vi "onDestroy.vi"(8 "error in (no error)":errorcluster, 11 "Pump":refnum<class "Pump.lvclass">) -> (0 "error out":errorcluster, 3 "Pump out":refnum<class "Pump.lvclass">)   [LabVIEW 2014, in "Pump.lvclass"]
doc: "JKI State Machine Objects (SMO) 1.4.0.57\nJKI - JKI\nCopyright (c) 2018, JKI"
uses:
  Pump.lvclass
  Pump.lvclass/Pump.ctl
  <vilib>/JKI/JKI SMO/SMO/SMO.lvclass
panel:
  # "For instructions on how to use the JKI State Machine Objects, examples and video tutorials, visit:\nhttp://jki.net/state-machine-objects/\n\nJKI State Machine Objects™\nhttp://jki.net/state-machine-objects/\nCopyright (C) 2005-2015, JKI <info@jki.net>\nALL RIGHTS RESERVED"
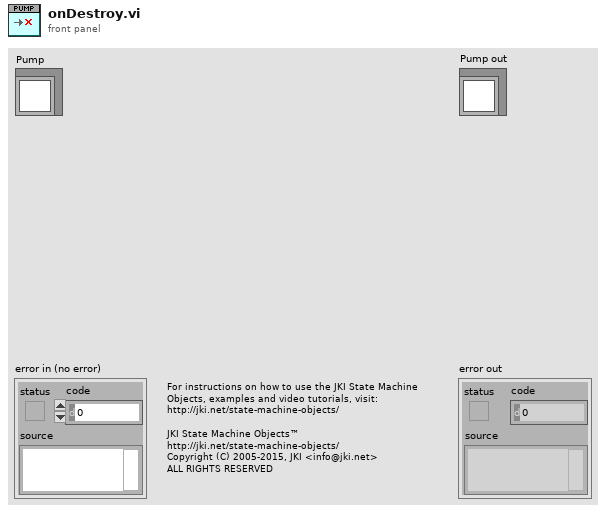
[diagram p1: front panel]
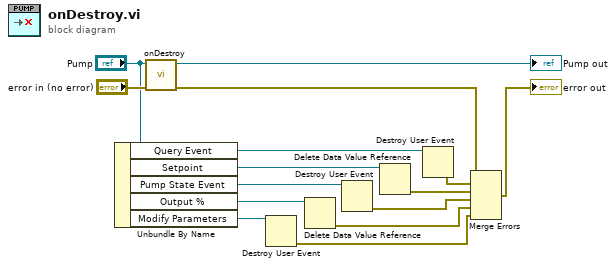
[diagram p0: block diagram]
diagram:
  n1 = Unbundle By Name("Pump") -> ("Query Event"=w12:refnum<user-event>, "Setpoint"=w7:refnum<data-value>, "Pump State Event"=w6:refnum<user-event>, "Output %"=w4:refnum<data-value>, "Modify Parameters"=w2:refnum<user-event>)
  n2 = call-parent "onDestroy.vi"("error in (no error)"="error in (no error)", "SMO"="Pump") -> ("error out"=w10:errorcluster, "SMO out"=→"Pump out":refnum<class "Pump.lvclass">)  [unwired: 8 in]
  n3 = Destroy User Event(user event=w2) -> (error out=w1:errorcluster)  [unwired: 1 in]
  n4 = Delete Data Value Reference(data value reference=w4) -> (error out=w3:errorcluster)  [unwired: 1 in, 1 out]
  n5 = Destroy User Event(user event=w6) -> (error out=w5:errorcluster)  [unwired: 1 in]
  n6 = Delete Data Value Reference(data value reference=w7) -> (error out=w8:errorcluster)  [unwired: 1 in, 1 out]
  n7 = Destroy User Event(user event=w12) -> (error out=w11:errorcluster)  [unwired: 1 in]
  n8 = Merge Errors(w10, w11, w8, w5, w3, w1) -> (→"error out":errorcluster)
